vi "fgv_Znorm_d4app.vi"(7 "Function":enum16{"Idle", "Write", "Read"}(ring), 8 "error in (no error)":errorcluster, 9 "Znorm_um_Scaling":dbl, 10 "acceptance angle":dbl, 11 "xyzNormalizedCoordinates":T1={"XYZ Start"=[{"X"=0.0, "Y"=0.0, "Z"=0.0}], "XYZ Stop"=[]}) -> (0 "error out":errorcluster, 2 "E Field":string[](array[string]), 3 "Phase Field":string[](array[string]))   [LabVIEW 2020]
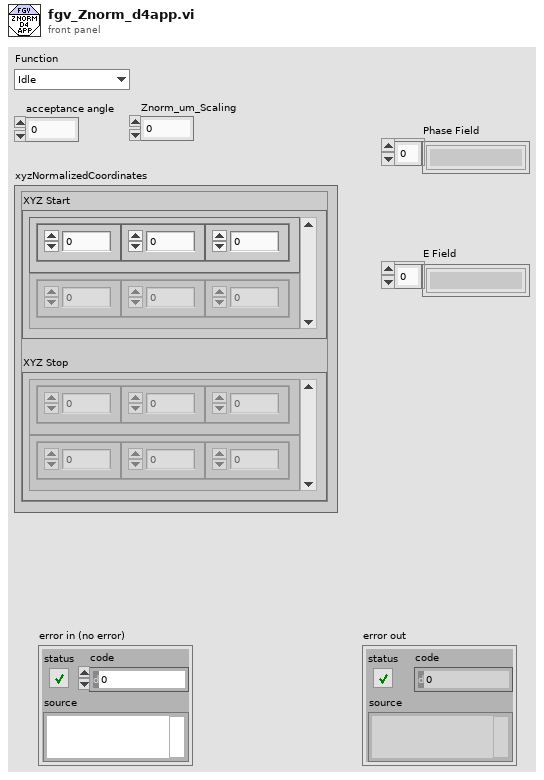
[diagram p1: front panel]
types:
  T1 = cluster{"XYZ Start":cluster{"X":sgl, "Y":sgl, "Z":sgl}[], "XYZ Stop":cluster{"X":sgl, "Y":sgl, "Z":sgl}[]}
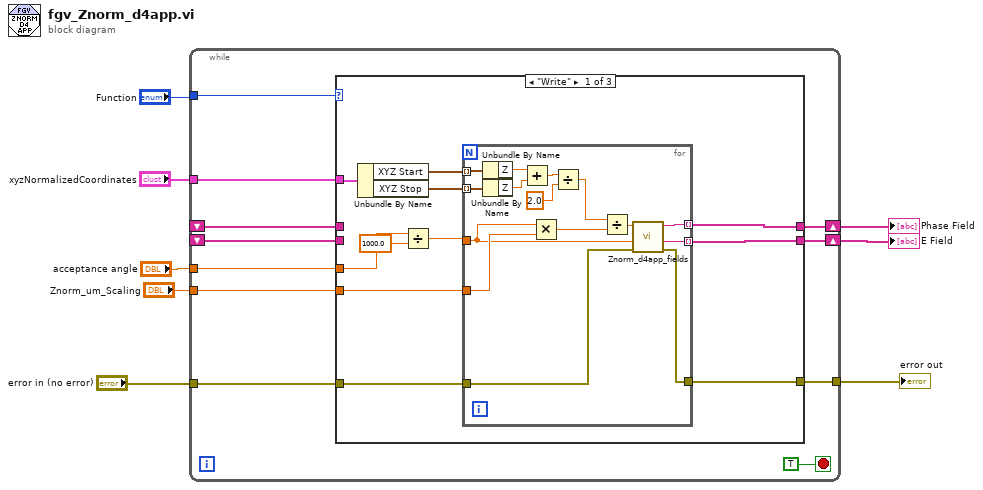
[diagram p0: block diagram]
diagram:
  n1 = while {
    tunnel: "Function" -> [w18]
    shift-right: [w16] -> w7
    shift-left: _ -> [w17]
    shift-right: [w14] -> w6
    shift-left: _ -> [w15]
    tunnel: "xyzNormalizedCoordinates" -> [w13]
    tunnel: "acceptance angle" -> [w12]
    tunnel: "Znorm_um_Scaling" -> [w11]
    tunnel: "error in (no error)" -> [w10]
    tunnel: [w9] -> w1
    stop <- TRUE stop-if-true
    n2 = case shown="\"Write\"" w18 {
      tunnel: w17 -> [_ w48 _]
      tunnel: [w29 w48 _] -> w16
      tunnel: w15 -> [_ w47 _]
      tunnel: [w30 w47 _] -> w14
      tunnel: w13 -> [w28 _ _]
      tunnel: w12 -> [w22 _ _]
      tunnel: w11 -> [w25 _ _]
      tunnel: w10 -> [w24 w46 w49]
      tunnel: [w23 w46 w49] -> w9
      frame "Write" {
        n3 = Unbundle By Name(w28) -> ("XYZ Start"=w27:cluster{"X":sgl, "Y":sgl, "Z":sgl}[], "XYZ Stop"=w26:cluster{"X":sgl, "Y":sgl, "Z":sgl}[])
        n4 = Divide(x=w22, y=1000.0) -> (x/y=w21:dbl)
        n5 = for {
          tunnel: [w45] -> w30 mode=indexing
          tunnel: [w44] -> w29 mode=indexing
          tunnel: w27 -> [w43] mode=indexing
          tunnel: w26 -> [w42] mode=indexing
          tunnel: w21 -> [w35]
          tunnel: w25 -> [w36]
          tunnel: w24 -> [w32]
          tunnel: [w31] -> w23
          n6 = Unbundle By Name(w43) -> ("Z"=w41:sgl)
          n7 = Unbundle By Name(w42) -> ("Z"=w40:sgl)
          n8 = Add(x=w41, y=w40) -> (x+y=w39:sgl)
          n9 = Multiply(x=w35, y=w36) -> (x*y=w34:dbl)
          n10 = Divide(x=w39, y=sgl 2.0) -> (x/y=w37:sgl)
          n11 = Divide(x=w37, y=w34) -> (x/y=w33:dbl)
          n12 = call "Znorm_d4app_fields.vi"("error in (no error)"=w32, "acceptance angle"=w35, "Zn"=w33) -> ("error out"=w31:errorcluster, "E field"=w45:string, "Phase Field"=w44:string)  [unwired: 6 in]
        }
      }
      frame "Read" {
      }
      frame "Idle", Default {
      }
    }
  }
  "E Field" <- w6
  "Phase Field" <- w7
  "error out" <- w1
